vi "ComparableVersionString.vi"(11 "Version in":string) -> (3 "Version as comparable":string)   [LabVIEW 2019, in "ByteLVDevEnv.lvlib"]
uses:
  ByteLVDevEnv.lvlib
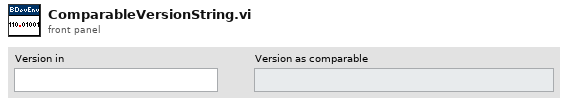
[diagram p1: front panel]
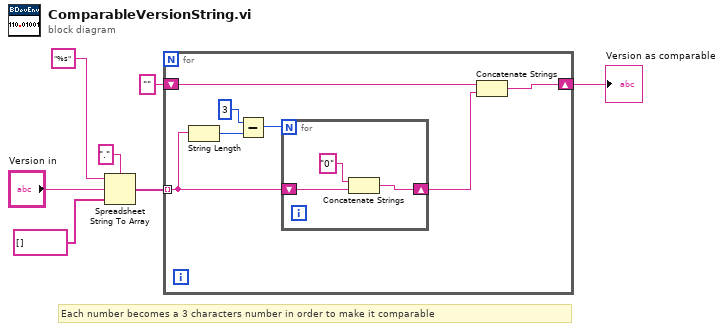
[diagram p0: block diagram]
diagram:
  # "Each number becomes a 3 characters number in order to make it comparable"
  n1 = Spreadsheet String To Array(delimiter (Tab)=".", format string="%s", spreadsheet string="Version in", array type (2D Dbl)=string[] []) -> (array=w4:string[])
  n2 = for {
    tunnel: w4 -> [w13] mode=indexing
    shift-right: [w10] -> w1
    shift-left: "" -> [w8]
    n3 = String Length(string=w13) -> (length=w14:i32)
    n4 = Subtract(x=3 ("y"), y=w14) -> (x-y=w12:i32)
    n5 = for {
      N: w12 -> [_]
      shift-right: [w16] -> w9
      shift-left: w13 -> [w17]
      n6 = Concatenate Strings("0" ("string"), w17) -> (w16:string)
    }
    n7 = Concatenate Strings(w8, w9) -> (w10:string)
  }
  "Version as comparable" <- w1
